vi "PathPlanner_Path_BezierToWaypoints.vi"(11 "BezierPoints":T2[](array[typedef]) {"Y" format="%14.3f"; "X" format="%14.3f"}) -> (3 "Waypoints":T1[](array[typedef]) {"nextControl"."Y" format="%14.3f"; "nextControl"."X" format="%14.3f"; "anchor"."Y" format="%14.3f"; "anchor"."X" format="%14.3f"; "prevControl"."Y" format="%14.3f"; "prevControl"."X" format="%14.3f"})   [LabVIEW 2019, in "PathPlanner24.lvlib"]
doc: "Convert bezier points to waypoints allowing them to be written to a JSON string or used to create Paths.\n\nInputs: \n - Bezier - array of translation2s - List of bezier points\n\nOutputs:\n - waypoints - array of cluster - waypoints compatible with pathplanner path JSON strings."
uses:
  PathPlanner24.lvlib
  TypeDef/PathPlannerWaypoint.ctl
  <vilib>/Rock Robotics/WPI/ThirdParty/JAS_Junk/TrajLib/TypeDef/TRANSLATION2D.ctl
  <vilib>/Rock Robotics/WPI/ThirdParty/JAS_Junk/TrajLib/Trajectory_Library.lvlib
panel:
  in  "waypoints":T1={"prevControl"={"X"=1e+30, "Y"=1e+31}, "anchor"={"X"=1e+30, "Y"=1e+31}, "nextControl"={"X"=1e+30, "Y"=1e+31}, "PrevExists"=FALSE, "NextExists"=FALSE} {"nextControl"."Y" format="%14.3f"; "nextControl"."X" format="%14.3f"; "anchor"."Y" format="%14.3f"; "anchor"."X" format="%14.3f"; "prevControl"."Y" format="%14.3f"; "prevControl"."X" format="%14.3f"}
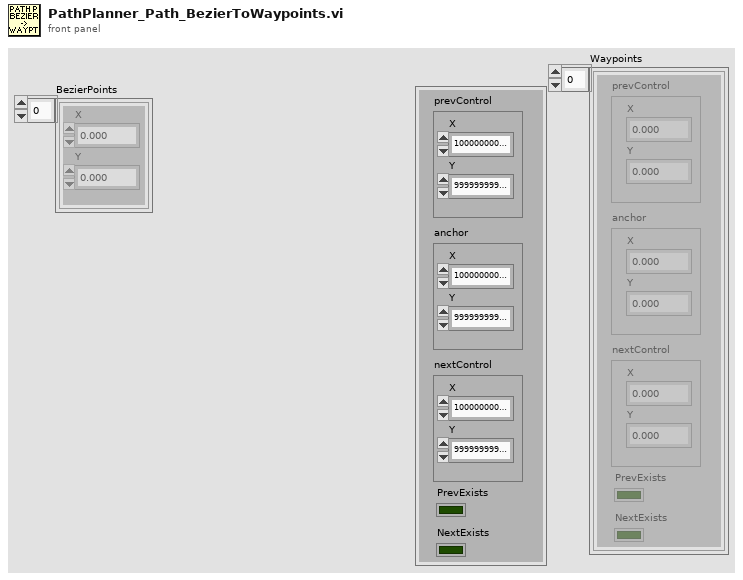
[diagram p1: front panel]
types:
  T1 = typedef "PathPlanner24.lvlib/PathPlannerWaypoint.ctl" = cluster{"prevControl":T2, "anchor":T2, "nextControl":T2, "PrevExists":bool, "NextExists":bool}
  T2 = typedef "Trajectory_Library.lvlib/TRANSLATION2D.ctl" = cluster{"X":dbl, "Y":dbl}
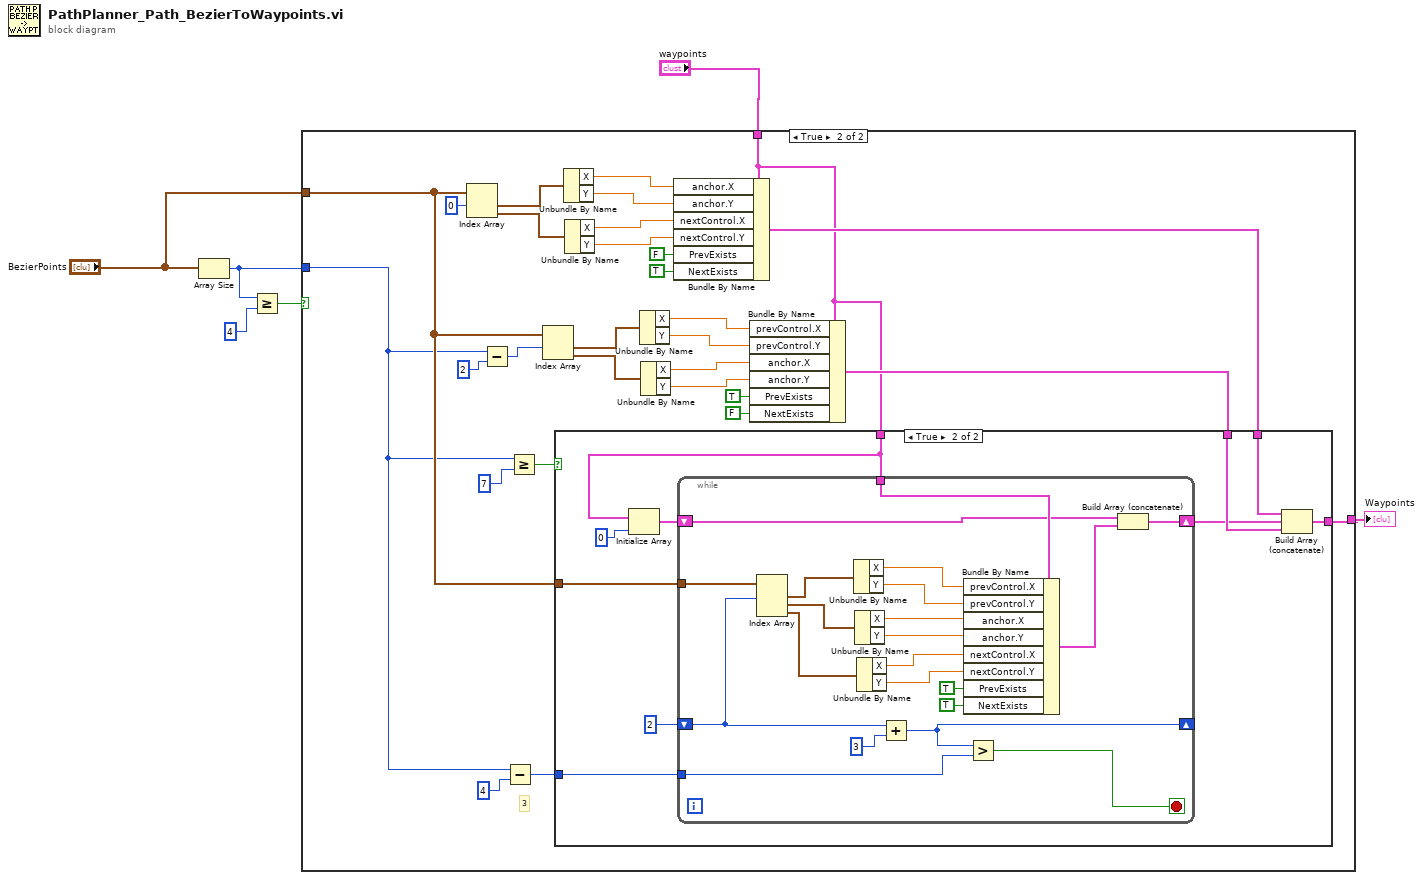
[diagram p0: block diagram]
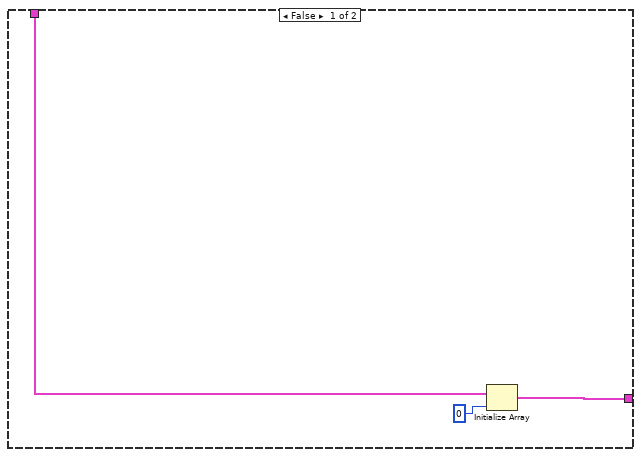
[diagram p2: hidden frame]
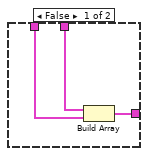
[diagram p3: hidden frame]
diagram:
  n1 = Array Size(array="BezierPoints") -> (size(s)=w2:i32)
  n2 = Greater Or Equal?(x=w2, y=4) -> (x >= y?=w3:bool)
  n3 = case shown="True" w3 {
    tunnel: "waypoints" -> [w8 w18]
    tunnel: "BezierPoints" -> [_ w17]
    tunnel: w2 -> [_ w16]
    tunnel: [w7 w19] -> w1
    frame False {
      n4 = Initialize Array(w8, 0 ("dimension size")) -> (w7:T1[])
    }
    frame True {
      # "3"
      n5 = Index Array(array=w17, index #1=0 ("index")) -> (element #1=w37:T2, element #2=w36:T2)  [unwired: 1 in]
      n6 = Subtract(x=w16, y=2) -> (x-y=w24:i32)
      n7 = Subtract(x=w16, y=4) -> (x-y=w14:i32)
      n8 = Greater Or Equal?(x=w16, y=7) -> (x >= y?=w22:bool)
      n9 = Index Array(array=w17, index #1=w24) -> (element #1=w31:T2, element #2=w30:T2)  [unwired: 1 in]
      n10 = Unbundle By Name(w37) -> ("X"=w35:dbl, "Y"=w34:dbl)
      n11 = Unbundle By Name(w36) -> ("X"=w33:dbl, "Y"=w32:dbl)
      n12 = Unbundle By Name(w31) -> ("X"=w29:dbl, "Y"=w28:dbl)
      n13 = Unbundle By Name(w30) -> ("X"=w27:dbl, "Y"=w26:dbl)
      n14 = Bundle By Name(cluster=w18, "anchor.X"=w35, "anchor.Y"=w34, "nextControl.X"=w33, "nextControl.Y"=w32, "PrevExists"=FALSE, "NextExists"=TRUE) -> (w21:T1)
      n15 = Bundle By Name(cluster=w18, "prevControl.X"=w29, "prevControl.Y"=w28, "anchor.X"=w27, "anchor.Y"=w26, "PrevExists"=TRUE, "NextExists"=FALSE) -> (w20:T1)
      n16 = case shown="True" w22 {
        tunnel: w21 -> [w41 w44]
        tunnel: w20 -> [w40 w43]
        tunnel: [w39 w45] -> w19
        tunnel: w18 -> [_ w48]
        tunnel: w17 -> [_ w47]
        tunnel: w14 -> [_ w46]
        frame False {
          n17 = Build Array(w41, w40) -> (w39:T1[])
        }
        frame True {
          n18 = Initialize Array(w48, 0 ("dimension size")) -> (w49:T1[])
          n19 = while {
            shift-right: [w57] -> _
            shift-left: 2 ("y") -> [w59]
            shift-right: [w54] -> w42
            shift-left: w49 -> [w61]
            tunnel: w48 -> [w72]
            tunnel: w47 -> [w71]
            tunnel: w46 -> [w56]
            stop <- w55 stop-if-true
            n20 = Index Array(array=w71, index #1=w59) -> (element #1=w70:T2, element #2=w69:T2, element #3=w68:T2)  [unwired: 2 in]
            n21 = Unbundle By Name(w70) -> ("X"=w67:dbl, "Y"=w66:dbl)
            n22 = Unbundle By Name(w69) -> ("X"=w65:dbl, "Y"=w64:dbl)
            n23 = Unbundle By Name(w68) -> ("X"=w63:dbl, "Y"=w62:dbl)
            n24 = Add(x=w59, y=3) -> (x+y=w57:i32)
            n25 = Bundle By Name(cluster=w72, "prevControl.X"=w67, "prevControl.Y"=w66, "anchor.X"=w65, "anchor.Y"=w64, "nextControl.X"=w63, "nextControl.Y"=w62, "PrevExists"=TRUE, "NextExists"=TRUE) -> (w60:T1)
            n26 = Greater?(x=w57, y=w56) -> (0:w55:bool)
            n27 = Build Array (concatenate)(w61, w60) -> (w54:T1[])
          }
          n28 = Build Array (concatenate)(w44, w42, w43) -> (w45:T1[])
        }
      }
    }
  }
  "Waypoints" <- w1
